vi "SeqEditor_StepMLSTcopy.vi"(8 "error in (no error)":errorcluster, 11 "NLTest in":refnum<class "NLTest.lvclass">) -> (0 "error out":errorcluster, 3 "NLTest out":refnum<class "NLTest.lvclass">)   [LabVIEW 2017, in "NLTest.lvclass"]
uses:
  NLTest.lvclass
  NLTest.lvclass/NLTest.ctl
  f15116b3-c504-4477-bb32-58f8fefe0bac.vi
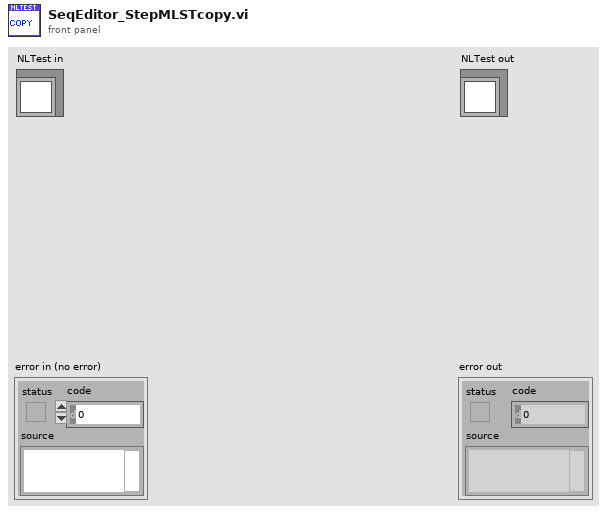
[diagram p1: front panel]
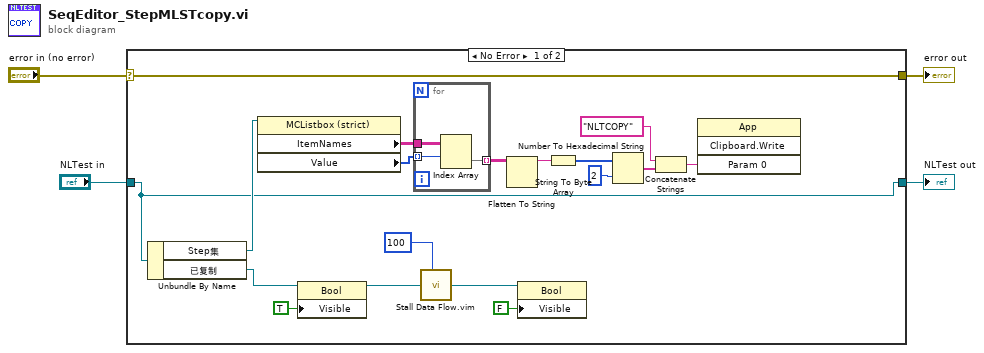
[diagram p0: block diagram]
diagram:
  n1 = case shown="No Error" "error in (no error)" {
    selector: "error in (no error)" -> [w22 w27]
    tunnel: [w22 w27] -> w3
    tunnel: [w20 w26] -> w1
    tunnel: "NLTest in" -> [w20 w26]
    frame No Error {
      n2 = Unbundle By Name(w20) -> ("Step集"=w21:refnum<vi>, "已复制"=w10:refnum<vi>)
      n3 = property class="MCListbox (strict)"(reference=w21) -> ("ItemNames"=w18:string[][], "Value"=w19:i32[])  [unwired: 1 in, 2 out]
      n4 = property class="Bool"(reference=w10, "Visible"=TRUE) -> (reference out=w7:refnum<vi>)  [unwired: 1 in, 1 out]
      n5 = for {
        tunnel: w19 -> [w24] mode=indexing
        tunnel: w18 -> [w25]
        tunnel: [w23] -> w17 mode=indexing
        n6 = Index Array(array=w25, index (row)=w24) -> (element=w23:string[])  [unwired: 1 in]
      }
      n7 = call "Stall Data Flow.vim"("value in"=w7, "milliseconds to wait"=u32 100) -> ("value out"=w6:refnum<vi>)  [unwired: 1 out]
      n8 = Flatten To String(anything=w17) -> (data string=w11:string)  [unwired: 3 in, 2 out]
      n9 = property class="Bool"(reference=w6, "Visible"=FALSE) -> ()  [unwired: 1 in, 2 out]
      n10 = String To Byte Array(string=w11) -> (unsigned byte array=w16:u8[])
      n11 = Number To Hexadecimal String(1:i16 2 ("width (-)"), 2:w16) -> (0:w12:string[])
      n12 = Concatenate Strings("NLTCOPY", w12) -> (w13:string)
      n13 = invoke class="App" method="Clipboard.Write"("Param 0"=w13) -> ()  [unwired: 3 in, 4 out]
    }
    frame Error {
    }
  }
  "error out" <- w3
  "NLTest out" <- w1
